vi "Send Error.vi"(8 "error in (no error)":errorcluster, 11 "Guardian in":refnum<class "Guardian.lvclass">) -> (0 "error out":errorcluster, 3 "Guardian out":refnum<class "Guardian.lvclass">)   [LabVIEW 2020, in "TALOS.lvlib" / "Guardian.lvlib" / "Guardian.lvclass"]
doc: "Use this VI to send an error to be processed by the Error Manager of the Distributed System.\n#What if the ASV update gives an error?"
uses:
  Guardian.lvclass
  Guardian.lvclass/Guardian.ctl
  Internal uServices/System uServices/Error Manager/Error Info.ctl
  Internal uServices/System uServices/Error Manager/Error Manager.lvclass
  TALOS.lvlib
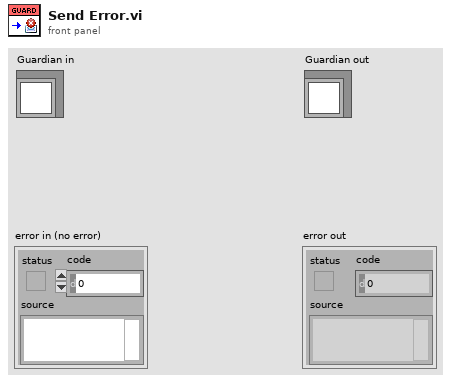
[diagram p1: front panel]
types:
  T1 = typedef "TALOS.lvlib/Error Manager.lvlib/Error Manager.lvclass/Error Info.ctl" = cluster{"error out":errorcluster, "Time Stamp":timestamp, "Machine Name":string, "GUID":string}
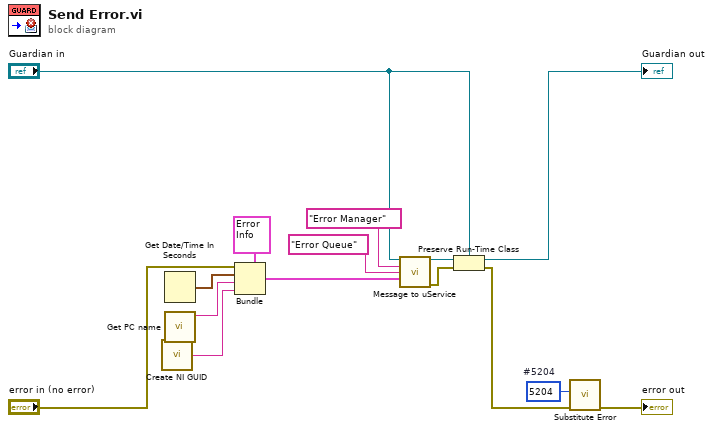
[diagram p0: block diagram]
diagram:
  w6 = 5204  # #5204
  n1 = call <vilib>:"Create NI GUID.vi"() -> ("NI GUID"=w11:string)
  n2 = Get Date/Time In Seconds() -> (seconds since 1Jan1904=w14:timestamp)
  n3 = call "Get PC name.vi"() -> ("Hostname"=w13:string)  [unwired: 10 in, 1 out]
  n4 = Bundle(cluster=T1 {"error out"={"status"=FALSE, "code"=0, "source"=""}, "Time Stamp"=timestamp(0 s since 1904-01-01), "Machine Name"="", "GUID"=""}, "error out"="error in (no error)", "Time Stamp"=w14, "Machine Name"=w13, "GUID"=w11) -> (w8:T1)
  n5 = call "Message to uService.vi"("Guardian in"="Guardian in", "uService ID"="Error Manager", "Message"="Error Queue", "Data"=w8) -> ("Guardian out"=w5:refnum<class "Guardian.lvclass">, "error out"=w1:errorcluster)  [unwired: 10 in]
  n6 = Preserve Run-Time Class(object in=w5, error in=w1, 2:"Guardian in") -> (object out=→"Guardian out":refnum<class "Guardian.lvclass">, error out=w2:errorcluster)
  n7 = call "Substitute Error.vi"("error in (no error)"=w2, "Error Code"=w6) -> ("error out"=→"error out":errorcluster)  [unwired: 9 in]
